vi "env chooser launcher.vi"(11 "launch time?":bool=TRUE) -> ()   [LabVIEW 2023]
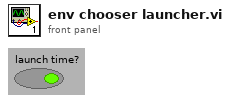
[diagram p1: front panel]
types:
  T1 = enum32{"Invalid", "Standard", "Closed", "Hidden", "Minimized", "Maximized"}
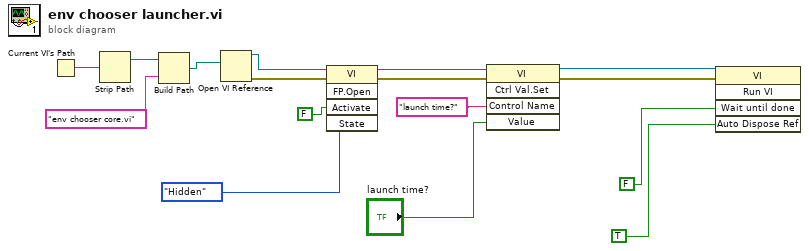
[diagram p0: block diagram]
diagram:
  n1 = Current VI's Path() -> (path=w12:path)
  n2 = Strip Path(path=w12) -> (stripped path=w7:path)  [unwired: 1 out]
  n3 = Build Path(base path=w7, name or relative path="env chooser core.vi") -> (appended path=w1:path)
  n4 = Open VI Reference(vi path=w1) -> (vi reference=w15:refnum<vi>, error out=w14:errorcluster)  [unwired: 5 in]
  n5 = invoke class="VI" method="FP.Open"(reference=w15, error in=w14, "Activate"=FALSE ("Wait Until Done"), "State"=T1."Hidden") -> (reference out=w5:refnum<vi>, error out=w6:errorcluster)  [unwired: 1 in, 3 out]
  n6 = invoke class="VI" method="Ctrl Val.Set"(reference=w5, "Control Name"="launch time?", "Value"="launch time?") -> (reference out=w4:refnum<vi>)  [unwired: 2 in, 4 out]
  n7 = invoke class="VI" method="Run VI"(reference=w4, error in=w6, "Wait until done"=FALSE ("Wait Until Done"), "Auto Dispose Ref"=TRUE ("Auto Dispose Reference")) -> ()  [unwired: 1 in, 5 out]
